vi "set TXP Resolution BandWidth.vi"(8 "error in (no error)":errorcluster, 10 "BW Value (Hz)":dbl format="%#_6p", 11 "Keysight 9020A in":refnum<class "Keysight 9020A.lvclass">) -> (0 "error out":errorcluster, 3 "Keysight 9020A out":refnum<class "Keysight 9020A.lvclass">)   [LabVIEW 2023, in "Spectrum Analyzer.lvlib" / "Keysight 9020A.lvclass"]
uses:
  Keysight 9020A.lvclass
  Keysight 9020A.lvclass/Keysight 9020A.ctl
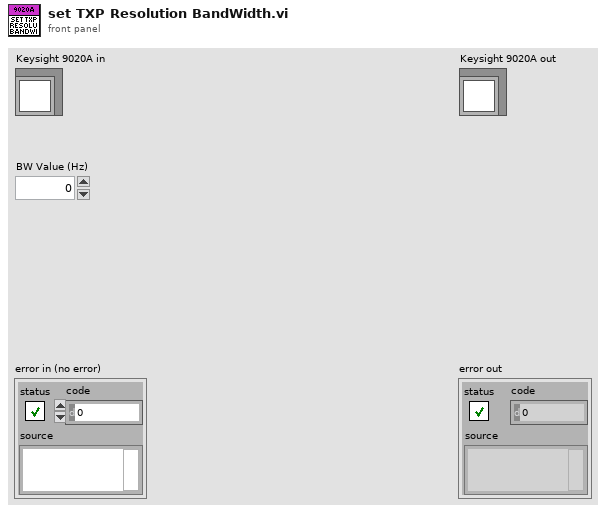
[diagram p1: front panel]
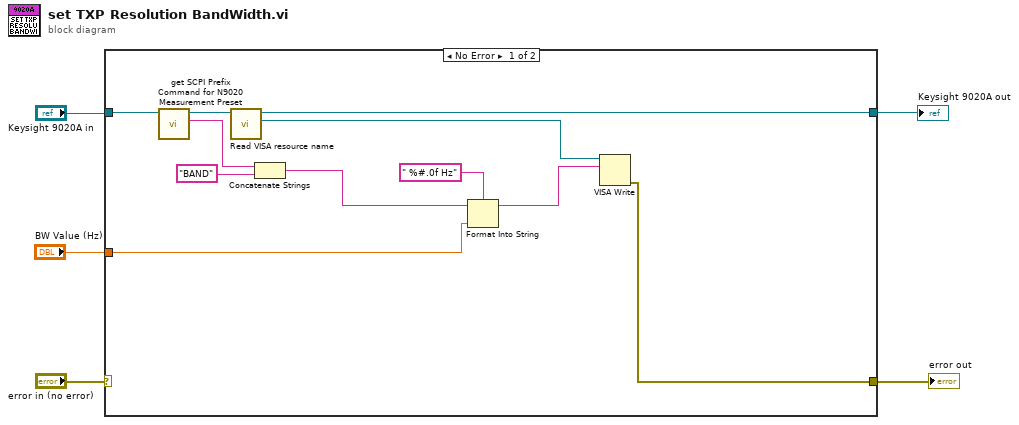
[diagram p0: block diagram]
diagram:
  n1 = case shown="No Error" "error in (no error)" {
    selector: "error in (no error)" -> [_ w17]
    tunnel: "Keysight 9020A in" -> [w10 w18]
    tunnel: [w16 w18] -> w5
    tunnel: [w12 w17] -> w1
    tunnel: "BW Value (Hz)" -> [w11 _]
    frame No Error {
      n2 = call "get SCPI Prefix Command for N9020 Measurement Preset.vi"("Keysight 9020A in"=w10) -> ("SCPI Prefix Command"=w8:string, "Keysight 9020A out"=w9:refnum<class "Keysight 9020A.lvclass">)  [unwired: 8 in, 1 out]
      n3 = call "Read VISA resource name.vi"("Keysight 9020A in"=w9) -> ("VISA resource name"=w15:refnum<visa-resource-name>, "Keysight 9020A out"=w16:refnum<class "Keysight 9020A.lvclass">)  [unwired: 8 in, 1 out]
      n4 = Concatenate Strings(w8, "BAND") -> (w6:string)
      n5 = Format Into String(format string=" %#.0f Hz", initial string=w6, w11) -> (resulting string=w14:string)  [unwired: 1 in, 1 out]
      n6 = VISA Write(VISA resource name=w15, write buffer=w14) -> (error out=w12:errorcluster)  [unwired: 1 in, 2 out]
    }
    frame Error {
    }
  }
  "error out" <- w1
  "Keysight 9020A out" <- w5
